vi "test data editor.vi"() -> ()   [LabVIEW 2019]
panel:
  out "standard error":string
  out "standard output":string
  out "error out 2":errorcluster
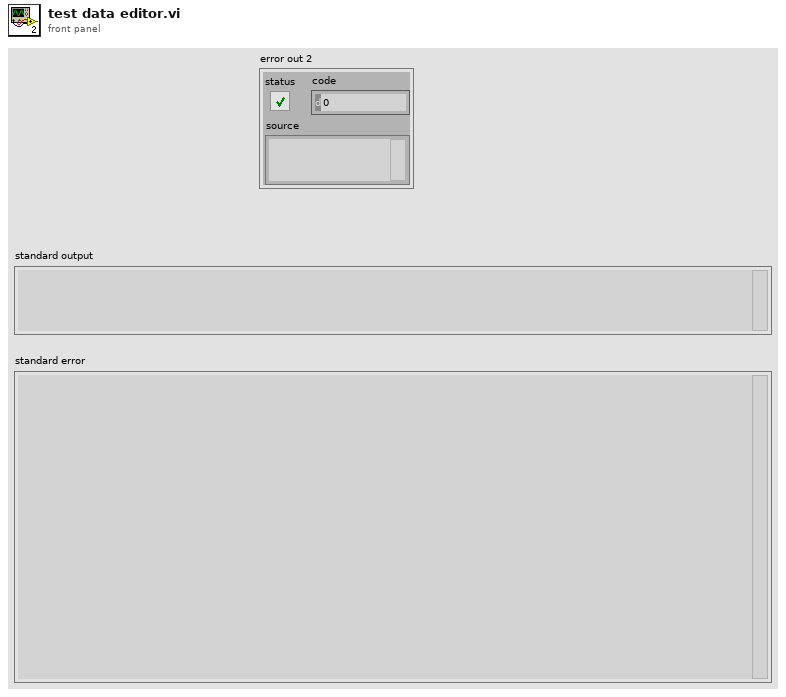
[diagram p1: front panel]
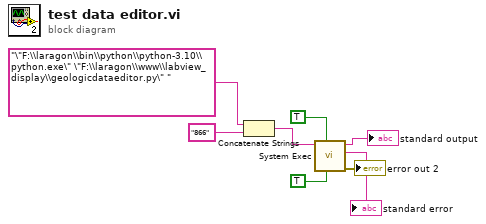
[diagram p0: block diagram]
diagram:
  n1 = Concatenate Strings("\"F:\\laragon\\bin\\python\\python-3.10\\python.exe\" \"F:\\laragon\\www\\labview_display\\geologicdataeditor.py\" " ("command line"), "866" ("string")) -> (w3:string)
  n2 = call <vilib>:"System Exec.vi"("run minimized? (F)"=TRUE, "wait until completion? (T)"=TRUE, "command line"=w3) -> ("error out"=→"error out 2":errorcluster, "standard error"=→"standard error":string, "standard output"=→"standard output":string)  [unwired: 5 in, 1 out]
